vi "Generate Sine Block.vi"(6 "amplitude":dbl=1.0, 7 "frequency":dbl=10.0, 8 "error in":errorcluster, 9 "sample rate":dbl=1000.0, 10 "start sample":dbl, 11 "samples":i32=100) -> (0 "error out":errorcluster, 2 "time":dbl[](array[numeric]), 3 "signal":dbl[](array[numeric]))   [LabVIEW 2026, in "Sine Generator.lvlib"]
doc: "Signal generation engine. Computes one block of a sine wave: signal[i] = amplitude * sin(2*pi*frequency*(start sample + i)/sample rate) and time[i] = i/sample rate in seconds, so every block starts at t = 0 on the time axis while the phase continues from the start sample. Amplitude is the peak value, frequency is in Hz and sample rate in S/s."
uses:
  Sine Generator.lvlib
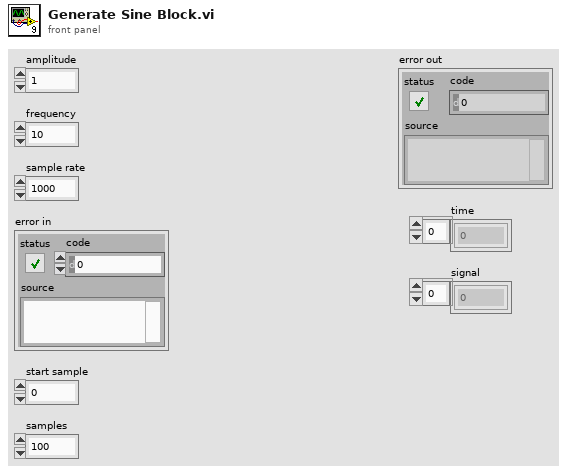
[diagram p1: front panel]
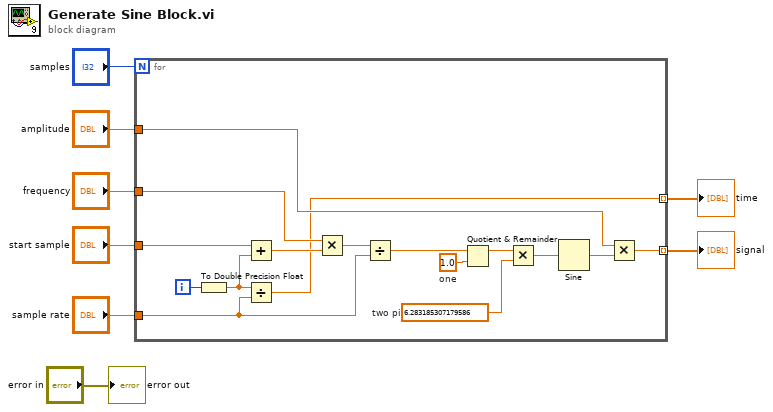
[diagram p0: block diagram]
diagram:
  n1 = for {
    N: "samples" -> [_]
    tunnel: "amplitude" -> [w15]
    tunnel: "frequency" -> [w23]
    tunnel: "sample rate" -> [w12]
    tunnel: "start sample" -> [w24]
    tunnel: [w11] -> w2 mode=indexing
    tunnel: [w10] -> w1 mode=indexing
    i -> [w9]
    w17 = 6.283185307179586  # two pi
    w19 = 1.0  # one
    n2 = To Double Precision Float(number=w9) -> (double precision float=w13:dbl)
    n3 = Add(x=w24, y=w13) -> (x+y=w22:dbl)
    n4 = Divide(x=w13, y=w12) -> (x/y=w11:dbl)
    n5 = Multiply(x=w23, y=w22) -> (x*y=w21:dbl)
    n6 = Divide(x=w21, y=w12) -> (x/y=w20:dbl)
    n7 = Quotient & Remainder(x=w20, y=w19) -> (x-y*floor(x/y)=w18:dbl)  [unwired: 1 out]
    n8 = Multiply(x=w18, y=w17) -> (x*y=w16:dbl)
    n9 = Sine(x=w16) -> (sin(x)=w14:dbl)
    n10 = Multiply(x=w15, y=w14) -> (x*y=w10:dbl)
  }
  "time" <- w2
  "signal" <- w1
  "error out" <- "error in"
